vi "Document_AddContent.vi"(8 "error in (no error)":errorcluster, 10 "Content":refnum<k24>, 11 "ooCalc in":refnum<class "ooCalc.lvclass">) -> (0 "error out":errorcluster, 3 "ooCalc out":refnum<class "ooCalc.lvclass">)   [LabVIEW 2009, in "ooCalc.lvclass"]
uses:
  ooCalc.lvclass
  C:/Projets/LAVAG/OpenOfficeRGT/AODL/DLLs/AODL.dll
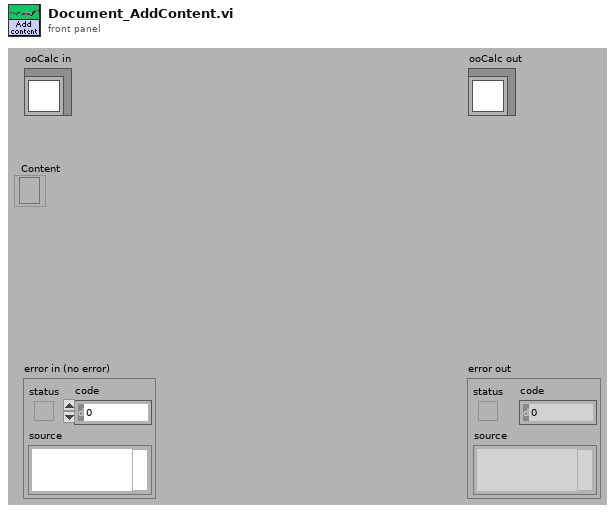
[diagram p1: front panel]
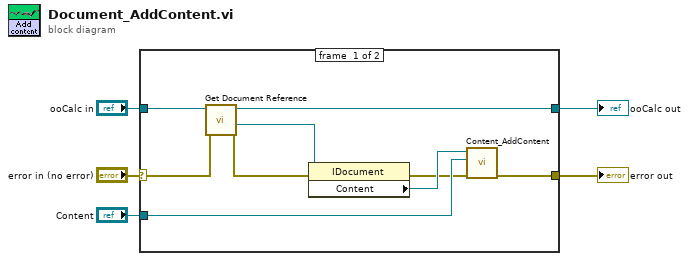
[diagram p0: block diagram]
diagram:
  n1 = case shown="No Error" "error in (no error)" {
    selector: "error in (no error)" -> [w7 w16]
    tunnel: [w11 w16] -> w5
    tunnel: [w8 w15] -> w3
    tunnel: "ooCalc in" -> [w9 w15]
    tunnel: "Content" -> [w13 _]
    frame #0 {
      n2 = call-dynamic "Get Document Reference.vi"("error in (no error)"=w7, "ooDocument in"=w9) -> ("error out"=w6:errorcluster, "Document"=w10:refnum<k24>, "ooDocument out"=w8:refnum<class "ooCalc.lvclass">)  [unwired: 7 in]
      n3 = property class="IDocument"(reference=w10, error in=w6) -> (error out=w12:errorcluster, "Content"=w14:refnum<k24>)  [unwired: 1 out]
      n4 = call "Content_AddContent.vi"("error in"=w12, "Content"=w13, "ContentCollection"=w14) -> ("error out"=w11:errorcluster)  [unwired: 7 in, 1 out]
    }
    frame #1 {
    }
  }
  "error out" <- w5
  "ooCalc out" <- w3
